vi "Correlation_Contrast_Tau_Manipulation.vi"(8 "Numeric 2":i32, 9 "Dont invert?":bool, 10 "Numeric":i32, 11 "MW Step Size":dbl=2e-09) -> (3 "Tau":dbl)   [LabVIEW 2024]
uses:
  <vilib>/Utility/error.llb/DialogTypeEnum.ctl
  SpinCore_API_file_location.vi
panel:
  in  "# of Instructions":u32=89
  in  "Instructions":T1(array[cluster])=[{"Instruct Data"=0, "Op Code"=0, "Flags"=[FALSE, FALSE, TRUE, FALSE, FALSE, FALSE, FALSE, TRUE, FALSE, FALSE, FALSE, FALSE, FALSE, FALSE, FALSE, FALSE, FALSE, FALSE, FALSE, FALSE, FALSE, FALSE, FALSE, TRUE], "Comments"="0 Triggers", "Time (s)"=1e-07}, {"Instruct Data"=0, "Op Code"=0, "Flags"=[FALSE, FALSE, FALSE, FALSE, FALSE, FALSE, FALSE, TRUE, FALSE, FALSE, FALSE, FALSE, FALSE, FALSE, FALSE, FALSE, FALSE, FALSE, FALSE, FALSE, FALSE, FALSE, FALSE, FALSE], "Comments"="1 Dark ", "Time (s)"=1e-05}, {"Instruct Data"=0, "Op Code"=0, "Flags"=[FALSE, FALSE, FALSE, FALSE, FALSE, FALSE, FALSE, TRUE, FALSE, FALSE, FALSE, FALSE, FALSE, FALSE, FALSE, FALSE, FALSE, FALSE, FALSE, FALSE, FALSE, FALSE, FALSE, FALSE], "Comments"="2 AOM Buffer", "Time (s)"=5e-07}, {"Instruct Data"=0, "Op Code"=0, "Flags"=[TRUE, FALSE, FALSE, TRUE, FALSE, FALSE, FALSE, TRUE, FALSE, FALSE, FALSE, FALSE, FALSE, FALSE, FALSE, FALSE, FALSE, FALSE, FALSE, FALSE, FALSE, FALSE, FALSE, FALSE], "Comments"="3 pi/2_X", "Time (s)"=3.7e-08}, {"Instruct Data"=0, "Op Code"=0, "Flags"=[FALSE, FALSE, FALSE, FALSE, FALSE, FALSE, FALSE, TRUE, FALSE, FALSE, FALSE, FALSE, FALSE, FALSE, FALSE, FALSE, FALSE, FALSE, FALSE, FALSE, FALSE, FALSE, FALSE, FALSE], "Comments"="4 tau/2", "Time (s)"=2.105e-06}, {"Instruct Data"=0, "Op Code"=0, "Flags"=[TRUE, FALSE, FALSE, TRUE, FALSE, FALSE, FALSE, TRUE, FALSE, FALSE, FALSE, FALSE, FALSE, FALSE, FALSE, FALSE, FALSE, FALSE, FALSE, FALSE, FALSE, FALSE, FALSE, FALSE], "Comments"="5  Pi_X", "Time (s)"=6.7e-08}, {"Instruct Data"=0, "Op Code"=0, "Flags"=[FALSE, FALSE, FALSE, FALSE, FALSE, FALSE, FALSE, TRUE, FALSE, FALSE, FALSE, FALSE, FALSE, FALSE, FALSE, FALSE, FALSE, FALSE, FALSE, FALSE, FALSE, FALSE, FALSE, FALSE], "Comments"="6 Tau", "Time (s)"=4.21e-06}, {"Instruct Data"=0, "Op Code"=0, "Flags"=[TRUE, FALSE, FALSE, FALSE, TRUE, FALSE, FALSE, TRUE, FALSE, FALSE, FALSE, FALSE, FALSE, FALSE, FALSE, FALSE, FALSE, FALSE, FALSE, FALSE, FALSE, FALSE, FALSE, FALSE], "Comments"="7 Pi_Y", "Time (s)"=7e-08}, {"Instruct Data"=0, "Op Code"=0, "Flags"=[FALSE, FALSE, FALSE, FALSE, FALSE, FALSE, FALSE, TRUE, FALSE, FALSE, FALSE, FALSE, FALSE, FALSE, FALSE, FALSE, FALSE, FALSE, FALSE, FALSE, FALSE, FALSE, FALSE, FALSE], "Comments"="8 Tau", "Time (s)"=4.21e-06}, {"Instruct Data"=0, "Op Code"=0, "Flags"=[TRUE, FALSE, FALSE, TRUE, FALSE, FALSE, FALSE, TRUE, FALSE, FALSE, FALSE, FALSE, FALSE, FALSE, FALSE, FALSE, FALSE, FALSE, FALSE, FALSE, FALSE, FALSE, FALSE, FALSE], "Comments"="9 Pi_X", "Time (s)"=6.7e-08}, {"Instruct Data"=0, "Op Code"=0, "Flags"=[FALSE, FALSE, FALSE, FALSE, FALSE, FALSE, FALSE, TRUE, FALSE, FALSE, FALSE, FALSE, FALSE, FALSE, FALSE, FALSE, FALSE, FALSE, FALSE, FALSE, FALSE, FALSE, FALSE, FALSE], "Comments"="10 tau", "Time (s)"=4.21e-06}, {"Instruct Data"=0, "Op Code"=0, "Flags"=[TRUE, FALSE, FALSE, FALSE, TRUE, FALSE, FALSE, TRUE, FALSE, FALSE, FALSE, FALSE, FALSE, FALSE, FALSE, FALSE, FALSE, FALSE, FALSE, FALSE, FALSE, FALSE, FALSE, FALSE], "Comments"="11 Pi_Y", "Time (s)"=7e-08}, {"Instruct Data"=0, "Op Code"=0, "Flags"=[FALSE, FALSE, FALSE, FALSE, FALSE, FALSE, FALSE, TRUE, FALSE, FALSE, FALSE, FALSE, FALSE, FALSE, FALSE, FALSE, FALSE, FALSE, FALSE, FALSE, FALSE, FALSE, FALSE, FALSE], "Comments"="12 Tau", "Time (s)"=4.21e-06}, {"Instruct Data"=0, "Op Code"=0, "Flags"=[TRUE, FALSE, FALSE, FALSE, TRUE, FALSE, FALSE, TRUE, FALSE, FALSE, FALSE, FALSE, FALSE, FALSE, FALSE, FALSE, FALSE, FALSE, FALSE, FALSE, FALSE, FALSE, FALSE, FALSE], "Comments"="13 Pi_Y", "Time (s)"=7e-08}, {"Instruct Data"=0, "Op Code"=0, "Flags"=[FALSE, FALSE, FALSE, FALSE, FALSE, FALSE, FALSE, TRUE, FALSE, FALSE, FALSE, FALSE, FALSE, FALSE, FALSE, FALSE, FALSE, FALSE, FALSE, FALSE, FALSE, FALSE, FALSE, FALSE], "Comments"="14 tau", "Time (s)"=4.21e-06}, {"Instruct Data"=0, "Op Code"=0, "Flags"=[TRUE, FALSE, FALSE, TRUE, FALSE, FALSE, FALSE, TRUE, FALSE, FALSE, FALSE, FALSE, FALSE, FALSE, FALSE, FALSE, FALSE, FALSE, FALSE, FALSE, FALSE, FALSE, FALSE, FALSE], "Comments"="15 Pi_X", "Time (s)"=6.7e-08}, {"Instruct Data"=0, "Op Code"=0, "Flags"=[FALSE, FALSE, FALSE, FALSE, FALSE, FALSE, FALSE, TRUE, FALSE, FALSE, FALSE, FALSE, FALSE, FALSE, FALSE, FALSE, FALSE, FALSE, FALSE, FALSE, FALSE, FALSE, FALSE, FALSE], "Comments"="16  tau", "Time (s)"=4.21e-06}, {"Instruct Data"=0, "Op Code"=0, "Flags"=[TRUE, FALSE, FALSE, FALSE, TRUE, FALSE, FALSE, TRUE, FALSE, FALSE, FALSE, FALSE, FALSE, FALSE, FALSE, FALSE, FALSE, FALSE, FALSE, FALSE, FALSE, FALSE, FALSE, FALSE], "Comments"="17 Pi_Y", "Time (s)"=7e-08}, {"Instruct Data"=0, "Op Code"=0, "Flags"=[FALSE, FALSE, FALSE, FALSE, FALSE, FALSE, FALSE, TRUE, FALSE, FALSE, FALSE, FALSE, FALSE, FALSE, FALSE, FALSE, FALSE, FALSE, FALSE, FALSE, FALSE, FALSE, FALSE, FALSE], "Comments"="18 tau", "Time (s)"=4.21e-06}, {"Instruct Data"=0, "Op Code"=0, "Flags"=[TRUE, FALSE, FALSE, TRUE, FALSE, FALSE, FALSE, TRUE, FALSE, FALSE, FALSE, FALSE, FALSE, FALSE, FALSE, FALSE, FALSE, FALSE, FALSE, FALSE, FALSE, FALSE, FALSE, FALSE], "Comments"="19 pi_X", "Time (s)"=6.7e-08}, {"Instruct Data"=0, "Op Code"=0, "Flags"=[FALSE, FALSE, FALSE, FALSE, FALSE, FALSE, FALSE, TRUE, FALSE, FALSE, FALSE, FALSE, FALSE, FALSE, FALSE, FALSE, FALSE, FALSE, FALSE, FALSE, FALSE, FALSE, FALSE, FALSE], "Comments"="20  tau/2", "Time (s)"=2.105e-06}, {"Instruct Data"=0, "Op Code"=0, "Flags"=[TRUE, FALSE, FALSE, FALSE, TRUE, FALSE, FALSE, TRUE, FALSE, FALSE, FALSE, FALSE, FALSE, FALSE, FALSE, FALSE, FALSE, FALSE, FALSE, FALSE, FALSE, FALSE, FALSE, FALSE], "Comments"="21 pi/2_Y", "Time (s)"=3.9e-08}, {"Instruct Data"=0, "Op Code"=0, "Flags"=[FALSE, FALSE, FALSE, FALSE, FALSE, FALSE, FALSE, TRUE, FALSE, FALSE, FALSE, FALSE, FALSE, FALSE, FALSE, FALSE, FALSE, FALSE, FALSE, FALSE, FALSE, FALSE, FALSE, FALSE], "Comments"="22 CC tau", "Time (s)"=1e-08}, {"Instruct Data"=0, "Op Code"=0, "Flags"=[TRUE, FALSE, FALSE, TRUE, FALSE, FALSE, FALSE, TRUE, FALSE, FALSE, FALSE, FALSE, FALSE, FALSE, FALSE, FALSE, FALSE, FALSE, FALSE, FALSE, FALSE, FALSE, FALSE, FALSE], "Comments"="23  pi/2_X", "Time (s)"=3.7e-08}, {"Instruct Data"=0, "Op Code"=0, "Flags"=[FALSE, FALSE, FALSE, FALSE, FALSE, FALSE, FALSE, TRUE, FALSE, FALSE, FALSE, FALSE, FALSE, FALSE, FALSE, FALSE, FALSE, FALSE, FALSE, FALSE, FALSE, FALSE, FALSE, FALSE], "Comments"="24  tau/2", "Time (s)"=2.105e-06}, {"Instruct Data"=0, "Op Code"=0, "Flags"=[TRUE, FALSE, FALSE, TRUE, FALSE, FALSE, FALSE, TRUE, FALSE, FALSE, FALSE, FALSE, FALSE, FALSE, FALSE, FALSE, FALSE, FALSE, FALSE, FALSE, FALSE, FALSE, FALSE, FALSE], "Comments"="25  pi_X", "Time (s)"=6.7e-08}, {"Instruct Data"=0, "Op Code"=0, "Flags"=[FALSE, FALSE, FALSE, FALSE, FALSE, FALSE, FALSE, TRUE, FALSE, FALSE, FALSE, FALSE, FALSE, FALSE, FALSE, FALSE, FALSE, FALSE, FALSE, FALSE, FALSE, FALSE, FALSE, FALSE], "Comments"="26  tau", "Time (s)"=4.21e-06}, {"Instruct Data"=0, "Op Code"=0, "Flags"=[TRUE, FALSE, FALSE, FALSE, TRUE, FALSE, FALSE, TRUE, FALSE, FALSE, FALSE, FALSE, FALSE, FALSE, FALSE, FALSE, FALSE, FALSE, FALSE, FALSE, FALSE, FALSE, FALSE, FALSE], "Comments"="27  pi_Y", "Time (s)"=7e-08}, {"Instruct Data"=0, "Op Code"=0, "Flags"=[FALSE, FALSE, FALSE, FALSE, FALSE, FALSE, FALSE, TRUE, FALSE, FALSE, FALSE, FALSE, FALSE, FALSE, FALSE, FALSE, FALSE, FALSE, FALSE, FALSE, FALSE, FALSE, FALSE, FALSE], "Comments"="28  tau", "Time (s)"=4.21e-06}, {"Instruct Data"=0, "Op Code"=0, "Flags"=[TRUE, FALSE, FALSE, TRUE, FALSE, FALSE, FALSE, TRUE, FALSE, FALSE, FALSE, FALSE, FALSE, FALSE, FALSE, FALSE, FALSE, FALSE, FALSE, FALSE, FALSE, FALSE, FALSE, FALSE], "Comments"="29  Pi_X", "Time (s)"=6.7e-08}, {"Instruct Data"=0, "Op Code"=0, "Flags"=[FALSE, FALSE, FALSE, FALSE, FALSE, FALSE, FALSE, TRUE, FALSE, FALSE, FALSE, FALSE, FALSE, FALSE, FALSE, FALSE, FALSE, FALSE, FALSE, FALSE, FALSE, FALSE, FALSE, FALSE], "Comments"="30  tau", "Time (s)"=4.21e-06}, {"Instruct Data"=0, "Op Code"=0, "Flags"=[TRUE, FALSE, FALSE, FALSE, TRUE, FALSE, FALSE, TRUE, FALSE, FALSE, FALSE, FALSE, FALSE, FALSE, FALSE, FALSE, FALSE, FALSE, FALSE, FALSE, FALSE, FALSE, FALSE, FALSE], "Comments"="31  Pi_y", "Time (s)"=7e-08}, {"Instruct Data"=0, "Op Code"=0, "Flags"=[FALSE, FALSE, FALSE, FALSE, FALSE, FALSE, FALSE, TRUE, FALSE, FALSE, FALSE, FALSE, FALSE, FALSE, FALSE, FALSE, FALSE, FALSE, FALSE, FALSE, FALSE, FALSE, FALSE, FALSE], "Comments"="32  tau", "Time (s)"=4.21e-06}, {"Instruct Data"=0, "Op Code"=0, "Flags"=[TRUE, FALSE, FALSE, FALSE, TRUE, FALSE, FALSE, TRUE, FALSE, FALSE, FALSE, FALSE, FALSE, FALSE, FALSE, FALSE, FALSE, FALSE, FALSE, FALSE, FALSE, FALSE, FALSE, FALSE], "Comments"="33  Pi_Y", "Time (s)"=7e-08}, {"Instruct Data"=0, "Op Code"=0, "Flags"=[FALSE, FALSE, FALSE, FALSE, FALSE, FALSE, FALSE, TRUE, FALSE, FALSE, FALSE, FALSE, FALSE, FALSE, FALSE, FALSE, FALSE, FALSE, FALSE, FALSE, FALSE, FALSE, FALSE, FALSE], "Comments"="34  tau", "Time (s)"=4.21e-06}, {"Instruct Data"=0, "Op Code"=0, "Flags"=[TRUE, FALSE, FALSE, TRUE, FALSE, FALSE, FALSE, TRUE, FALSE, FALSE, FALSE, FALSE, FALSE, FALSE, FALSE, FALSE, FALSE, FALSE, FALSE, FALSE, FALSE, FALSE, FALSE, FALSE], "Comments"="35 Pi_X", "Time (s)"=6.7e-08}, {"Instruct Data"=0, "Op Code"=0, "Flags"=[FALSE, FALSE, FALSE, FALSE, FALSE, FALSE, FALSE, TRUE, FALSE, FALSE, FALSE, FALSE, FALSE, FALSE, FALSE, FALSE, FALSE, FALSE, FALSE, FALSE, FALSE, FALSE, FALSE, FALSE], "Comments"="36  tau", "Time (s)"=4.21e-06}, {"Instruct Data"=0, "Op Code"=0, "Flags"=[TRUE, FALSE, FALSE, FALSE, TRUE, FALSE, FALSE, TRUE, FALSE, FALSE, FALSE, FALSE, FALSE, FALSE, FALSE, FALSE, FALSE, FALSE, FALSE, FALSE, FALSE, FALSE, FALSE, FALSE], "Comments"="37  Pi_Y", "Time (s)"=7e-08}, {"Instruct Data"=0, "Op Code"=0, "Flags"=[FALSE, FALSE, FALSE, FALSE, FALSE, FALSE, FALSE, TRUE, FALSE, FALSE, FALSE, FALSE, FALSE, FALSE, FALSE, FALSE, FALSE, FALSE, FALSE, FALSE, FALSE, FALSE, FALSE, FALSE], "Comments"="38  tau", "Time (s)"=4.21e-06}, {"Instruct Data"=0, "Op Code"=0, "Flags"=[TRUE, FALSE, FALSE, TRUE, FALSE, FALSE, FALSE, TRUE, FALSE, FALSE, FALSE, FALSE, FALSE, FALSE, FALSE, FALSE, FALSE, FALSE, FALSE, FALSE, FALSE, FALSE, FALSE, FALSE], "Comments"="39  Pi_X", "Time (s)"=6.7e-08}, {"Instruct Data"=0, "Op Code"=0, "Flags"=[FALSE, FALSE, FALSE, FALSE, FALSE, FALSE, FALSE, TRUE, FALSE, FALSE, FALSE, FALSE, FALSE, FALSE, FALSE, FALSE, FALSE, FALSE, FALSE, FALSE, FALSE, FALSE, FALSE, FALSE], "Comments"="40  tau/2", "Time (s)"=2.105e-06}, {"Instruct Data"=0, "Op Code"=0, "Flags"=[TRUE, FALSE, FALSE, FALSE, TRUE, FALSE, FALSE, TRUE, FALSE, FALSE, FALSE, FALSE, FALSE, FALSE, FALSE, FALSE, FALSE, FALSE, FALSE, FALSE, FALSE, FALSE, FALSE, FALSE], "Comments"="41  pi/2_Y", "Time (s)"=3.9e-08}, {"Instruct Data"=0, "Op Code"=0, "Flags"=[FALSE, TRUE, FALSE, FALSE, FALSE, FALSE, FALSE, TRUE, FALSE, FALSE, FALSE, FALSE, FALSE, FALSE, FALSE, FALSE, FALSE, FALSE, FALSE, FALSE, FALSE, FALSE, FALSE, FALSE], "Comments"="42  AOM Buffer", "Time (s)"=5e-07}, {"Instruct Data"=0, "Op Code"=0, "Flags"=[FALSE, TRUE, FALSE, FALSE, FALSE, FALSE, FALSE, FALSE, FALSE, FALSE, FALSE, FALSE, FALSE, FALSE, FALSE, FALSE, FALSE, FALSE, FALSE, FALSE, FALSE, FALSE, FALSE, FALSE], "Comments"="43  inhibit off", "Time (s)"=5e-07}, {"Instruct Data"=0, "Op Code"=0, "Flags"=[FALSE, TRUE, FALSE, FALSE, FALSE, FALSE, FALSE, TRUE, FALSE, FALSE, FALSE, FALSE, FALSE, FALSE, FALSE, FALSE, FALSE, FALSE, FALSE, FALSE, FALSE, FALSE, FALSE, FALSE], "Comments"="44  AOM", "Time (s)"=5e-06}, {"Instruct Data"=0, "Op Code"=0, "Flags"=[FALSE, FALSE, FALSE, FALSE, FALSE, FALSE, FALSE, TRUE, FALSE, FALSE, FALSE, FALSE, FALSE, FALSE, FALSE, FALSE, FALSE, FALSE, FALSE, FALSE, FALSE, FALSE, FALSE, FALSE], "Comments"="45  AOM buffer", "Time (s)"=5e-07}, {"Instruct Data"=0, "Op Code"=0, "Flags"=[FALSE, FALSE, FALSE, FALSE, FALSE, FALSE, FALSE, TRUE, FALSE, FALSE, FALSE, FALSE, FALSE, FALSE, FALSE, FALSE, FALSE, FALSE, FALSE, FALSE, FALSE, FALSE, FALSE, FALSE], "Comments"="46  Dark", "Time (s)"=1e-05}, {"Instruct Data"=0, "Op Code"=0, "Flags"=[TRUE, FALSE, FALSE, TRUE, FALSE, FALSE, FALSE, TRUE, FALSE, FALSE, FALSE, FALSE, FALSE, FALSE, FALSE, FALSE, FALSE, FALSE, FALSE, FALSE, FALSE, FALSE, FALSE, FALSE], "Comments"="47  pi/2_X", "Time (s)"=3.6e-08}, {"Instruct Data"=0, "Op Code"=0, "Flags"=[FALSE, FALSE, FALSE, FALSE, FALSE, FALSE, FALSE, TRUE, FALSE, FALSE, FALSE, FALSE, FALSE, FALSE, FALSE, FALSE, FALSE, FALSE, FALSE, FALSE, FALSE, FALSE, FALSE, FALSE], "Comments"="48  tau/2", "Time (s)"=2.105e-06}, {"Instruct Data"=0, "Op Code"=0, "Flags"=[TRUE, FALSE, FALSE, TRUE, FALSE, FALSE, FALSE, TRUE, FALSE, FALSE, FALSE, FALSE, FALSE, FALSE, FALSE, FALSE, FALSE, FALSE, FALSE, FALSE, FALSE, FALSE, FALSE, FALSE], "Comments"="49 Pi_X", "Time (s)"=6.7e-08}, {"Instruct Data"=0, "Op Code"=0, "Flags"=[FALSE, FALSE, FALSE, FALSE, FALSE, FALSE, FALSE, TRUE, FALSE, FALSE, FALSE, FALSE, FALSE, FALSE, FALSE, FALSE, FALSE, FALSE, FALSE, FALSE, FALSE, FALSE, FALSE, FALSE], "Comments"="50 tau", "Time (s)"=4.21e-06}, {"Instruct Data"=0, "Op Code"=0, "Flags"=[TRUE, FALSE, FALSE, FALSE, TRUE, FALSE, FALSE, TRUE, FALSE, FALSE, FALSE, FALSE, FALSE, FALSE, FALSE, FALSE, FALSE, FALSE, FALSE, FALSE, FALSE, FALSE, FALSE, FALSE], "Comments"="51 Pi_y", "Time (s)"=7e-08}, {"Instruct Data"=0, "Op Code"=0, "Flags"=[FALSE, FALSE, FALSE, FALSE, FALSE, FALSE, FALSE, TRUE, FALSE, FALSE, FALSE, FALSE, FALSE, FALSE, FALSE, FALSE, FALSE, FALSE, FALSE, FALSE, FALSE, FALSE, FALSE, FALSE], "Comments"="52 tau", "Time (s)"=4.21e-06}, {"Instruct Data"=0, "Op Code"=0, "Flags"=[TRUE, FALSE, FALSE, TRUE, FALSE, FALSE, FALSE, TRUE, FALSE, FALSE, FALSE, FALSE, FALSE, FALSE, FALSE, FALSE, FALSE, FALSE, FALSE, FALSE, FALSE, FALSE, FALSE, FALSE], "Comments"="53 pi_x", "Time (s)"=6.7e-08}, {"Instruct Data"=0, "Op Code"=0, "Flags"=[FALSE, FALSE, FALSE, FALSE, FALSE, FALSE, FALSE, TRUE, FALSE, FALSE, FALSE, FALSE, FALSE, FALSE, FALSE, FALSE, FALSE, FALSE, FALSE, FALSE, FALSE, FALSE, FALSE, FALSE], "Comments"="54 tau", "Time (s)"=4.21e-06}, {"Instruct Data"=0, "Op Code"=0, "Flags"=[TRUE, FALSE, FALSE, FALSE, TRUE, FALSE, FALSE, TRUE, FALSE, FALSE, FALSE, FALSE, FALSE, FALSE, FALSE, FALSE, FALSE, FALSE, FALSE, FALSE, FALSE, FALSE, FALSE, FALSE], "Comments"="55 Pi_Y", "Time (s)"=7e-08}, {"Instruct Data"=0, "Op Code"=0, "Flags"=[FALSE, FALSE, FALSE, FALSE, FALSE, FALSE, FALSE, TRUE, FALSE, FALSE, FALSE, FALSE, FALSE, FALSE, FALSE, FALSE, FALSE, FALSE, FALSE, FALSE, FALSE, FALSE, FALSE, FALSE], "Comments"="56 tau", "Time (s)"=4.21e-06}, {"Instruct Data"=0, "Op Code"=0, "Flags"=[TRUE, FALSE, FALSE, FALSE, TRUE, FALSE, FALSE, TRUE, FALSE, FALSE, FALSE, FALSE, FALSE, FALSE, FALSE, FALSE, FALSE, FALSE, FALSE, FALSE, FALSE, FALSE, FALSE, FALSE], "Comments"="57 Pi_y", "Time (s)"=7e-08}, {"Instruct Data"=0, "Op Code"=0, "Flags"=[FALSE, FALSE, FALSE, FALSE, FALSE, FALSE, FALSE, TRUE, FALSE, FALSE, FALSE, FALSE, FALSE, FALSE, FALSE, FALSE, FALSE, FALSE, FALSE, FALSE, FALSE, FALSE, FALSE, FALSE], "Comments"="58 tau", "Time (s)"=4.21e-06}, {"Instruct Data"=0, "Op Code"=0, "Flags"=[TRUE, FALSE, FALSE, TRUE, FALSE, FALSE, FALSE, TRUE, FALSE, FALSE, FALSE, FALSE, FALSE, FALSE, FALSE, FALSE, FALSE, FALSE, FALSE, FALSE, FALSE, FALSE, FALSE, FALSE], "Comments"="59 Pi_x", "Time (s)"=6.7e-08}, {"Instruct Data"=0, "Op Code"=0, "Flags"=[FALSE, FALSE, FALSE, FALSE, FALSE, FALSE, FALSE, TRUE, FALSE, FALSE, FALSE, FALSE, FALSE, FALSE, FALSE, FALSE, FALSE, FALSE, FALSE, FALSE, FALSE, FALSE, FALSE, FALSE], "Comments"="60 tau", "Time (s)"=4.21e-06}, {"Instruct Data"=0, "Op Code"=0, "Flags"=[TRUE, FALSE, FALSE, FALSE, TRUE, FALSE, FALSE, TRUE, FALSE, FALSE, FALSE, FALSE, FALSE, FALSE, FALSE, FALSE, FALSE, FALSE, FALSE, FALSE, FALSE, FALSE, FALSE, FALSE], "Comments"="61 Pi_y", "Time (s)"=7e-08}, {"Instruct Data"=0, "Op Code"=0, "Flags"=[FALSE, FALSE, FALSE, FALSE, FALSE, FALSE, FALSE, TRUE, FALSE, FALSE, FALSE, FALSE, FALSE, FALSE, FALSE, FALSE, FALSE, FALSE, FALSE, FALSE, FALSE, FALSE, FALSE, FALSE], "Comments"="62 tau", "Time (s)"=4.21e-06}, {"Instruct Data"=0, "Op Code"=0, "Flags"=[TRUE, FALSE, FALSE, TRUE, FALSE, FALSE, FALSE, TRUE, FALSE, FALSE, FALSE, FALSE, FALSE, FALSE, FALSE, FALSE, FALSE, FALSE, FALSE, FALSE, FALSE, FALSE, FALSE, FALSE], "Comments"="63 pi_X", "Time (s)"=6.7e-08}, {"Instruct Data"=0, "Op Code"=0, "Flags"=[FALSE, FALSE, FALSE, FALSE, FALSE, FALSE, FALSE, TRUE, FALSE, FALSE, FALSE, FALSE, FALSE, FALSE, FALSE, FALSE, FALSE, FALSE, FALSE, FALSE, FALSE, FALSE, FALSE, FALSE], "Comments"="64 Tau /2", "Time (s)"=2.105e-06}, {"Instruct Data"=0, "Op Code"=0, "Flags"=[TRUE, FALSE, FALSE, FALSE, TRUE, FALSE, FALSE, TRUE, FALSE, FALSE, FALSE, FALSE, FALSE, FALSE, FALSE, FALSE, FALSE, FALSE, FALSE, FALSE, FALSE, FALSE, FALSE, FALSE], "Comments"="65 pi/2_Y", "Time (s)"=3.8e-08}, {"Instruct Data"=0, "Op Code"=0, "Flags"=[FALSE, FALSE, FALSE, FALSE, FALSE, FALSE, FALSE, TRUE, FALSE, FALSE, FALSE, FALSE, FALSE, FALSE, FALSE, FALSE, FALSE, FALSE, FALSE, FALSE, FALSE, FALSE, FALSE, FALSE], "Comments"="66  TAU CC", "Time (s)"=1e-08}, {"Instruct Data"=0, "Op Code"=0, "Flags"=[TRUE, FALSE, FALSE, TRUE, FALSE, FALSE, FALSE, TRUE, FALSE, FALSE, FALSE, FALSE, FALSE, FALSE, FALSE, FALSE, FALSE, FALSE, FALSE, FALSE, FALSE, FALSE, FALSE, FALSE], "Comments"="67 pi/2_X", "Time (s)"=3.7e-08}, {"Instruct Data"=0, "Op Code"=0, "Flags"=[FALSE, FALSE, FALSE, FALSE, FALSE, FALSE, FALSE, TRUE, FALSE, FALSE, FALSE, FALSE, FALSE, FALSE, FALSE, FALSE, FALSE, FALSE, FALSE, FALSE, FALSE, FALSE, FALSE, FALSE], "Comments"="68 tau/2", "Time (s)"=2.105e-06}, {"Instruct Data"=0, "Op Code"=0, "Flags"=[TRUE, FALSE, FALSE, TRUE, FALSE, FALSE, FALSE, TRUE, FALSE, FALSE, FALSE, FALSE, FALSE, FALSE, FALSE, FALSE, FALSE, FALSE, FALSE, FALSE, FALSE, FALSE, FALSE, FALSE], "Comments"="69 Pi_x", "Time (s)"=6.7e-08}, {"Instruct Data"=0, "Op Code"=0, "Flags"=[FALSE, FALSE, FALSE, FALSE, FALSE, FALSE, FALSE, TRUE, FALSE, FALSE, FALSE, FALSE, FALSE, FALSE, FALSE, FALSE, FALSE, FALSE, FALSE, FALSE, FALSE, FALSE, FALSE, FALSE], "Comments"="70 tau", "Time (s)"=4.21e-06}, {"Instruct Data"=0, "Op Code"=0, "Flags"=[TRUE, FALSE, FALSE, FALSE, TRUE, FALSE, FALSE, TRUE, FALSE, FALSE, FALSE, FALSE, FALSE, FALSE, FALSE, FALSE, FALSE, FALSE, FALSE, FALSE, FALSE, FALSE, FALSE, FALSE], "Comments"="71 Pi_y", "Time (s)"=7e-08}, {"Instruct Data"=0, "Op Code"=0, "Flags"=[FALSE, FALSE, FALSE, FALSE, FALSE, FALSE, FALSE, TRUE, FALSE, FALSE, FALSE, FALSE, FALSE, FALSE, FALSE, FALSE, FALSE, FALSE, FALSE, FALSE, FALSE, FALSE, FALSE, FALSE], "Comments"="72 tau", "Time (s)"=4.21e-06}, {"Instruct Data"=0, "Op Code"=0, "Flags"=[TRUE, FALSE, FALSE, TRUE, FALSE, FALSE, FALSE, TRUE, FALSE, FALSE, FALSE, FALSE, FALSE, FALSE, FALSE, FALSE, FALSE, FALSE, FALSE, FALSE, FALSE, FALSE, FALSE, FALSE], "Comments"="73 Pi_x", "Time (s)"=6.7e-08}, {"Instruct Data"=0, "Op Code"=0, "Flags"=[FALSE, FALSE, FALSE, FALSE, FALSE, FALSE, FALSE, TRUE, FALSE, FALSE, FALSE, FALSE, FALSE, FALSE, FALSE, FALSE, FALSE, FALSE, FALSE, FALSE, FALSE, FALSE, FALSE, FALSE], "Comments"="74 tau", "Time (s)"=4.21e-06}, {"Instruct Data"=0, "Op Code"=0, "Flags"=[TRUE, FALSE, FALSE, FALSE, TRUE, FALSE, FALSE, TRUE, FALSE, FALSE, FALSE, FALSE, FALSE, FALSE, FALSE, FALSE, FALSE, FALSE, FALSE, FALSE, FALSE, FALSE, FALSE, FALSE], "Comments"="75 Pi_Y", "Time (s)"=7e-08}, {"Instruct Data"=0, "Op Code"=0, "Flags"=[FALSE, FALSE, FALSE, FALSE, FALSE, FALSE, FALSE, TRUE, FALSE, FALSE, FALSE, FALSE, FALSE, FALSE, FALSE, FALSE, FALSE, FALSE, FALSE, FALSE, FALSE, FALSE, FALSE, FALSE], "Comments"="76 tau ", "Time (s)"=4.21e-06}, {"Instruct Data"=0, "Op Code"=0, "Flags"=[TRUE, FALSE, FALSE, FALSE, TRUE, FALSE, FALSE, TRUE, FALSE, FALSE, FALSE, FALSE, FALSE, FALSE, FALSE, FALSE, FALSE, FALSE, FALSE, FALSE, FALSE, FALSE, FALSE, FALSE], "Comments"="77 Pi_y", "Time (s)"=7e-08}, {"Instruct Data"=0, "Op Code"=0, "Flags"=[FALSE, FALSE, FALSE, FALSE, FALSE, FALSE, FALSE, TRUE, FALSE, FALSE, FALSE, FALSE, FALSE, FALSE, FALSE, FALSE, FALSE, FALSE, FALSE, FALSE, FALSE, FALSE, FALSE, FALSE], "Comments"="78 tau", "Time (s)"=4.21e-06}, {"Instruct Data"=0, "Op Code"=0, "Flags"=[TRUE, FALSE, FALSE, TRUE, FALSE, FALSE, FALSE, TRUE, FALSE, FALSE, FALSE, FALSE, FALSE, FALSE, FALSE, FALSE, FALSE, FALSE, FALSE, FALSE, FALSE, FALSE, FALSE, FALSE], "Comments"="79 Pi_x", "Time (s)"=6.7e-08}, {"Instruct Data"=0, "Op Code"=0, "Flags"=[FALSE, FALSE, FALSE, FALSE, FALSE, FALSE, FALSE, TRUE, FALSE, FALSE, FALSE, FALSE, FALSE, FALSE, FALSE, FALSE, FALSE, FALSE, FALSE, FALSE, FALSE, FALSE, FALSE, FALSE], "Comments"="80 tau", "Time (s)"=4.21e-06}, {"Instruct Data"=0, "Op Code"=0, "Flags"=[TRUE, FALSE, FALSE, FALSE, TRUE, FALSE, FALSE, TRUE, FALSE, FALSE, FALSE, FALSE, FALSE, FALSE, FALSE, FALSE, FALSE, FALSE, FALSE, FALSE, FALSE, FALSE, FALSE, FALSE], "Comments"="81 Pi_y", "Time (s)"=7e-08}, {"Instruct Data"=0, "Op Code"=0, "Flags"=[FALSE, FALSE, FALSE, FALSE, FALSE, FALSE, FALSE, TRUE, FALSE, FALSE, FALSE, FALSE, FALSE, FALSE, FALSE, FALSE, FALSE, FALSE, FALSE, FALSE, FALSE, FALSE, FALSE, FALSE], "Comments"="82 tau", "Time (s)"=4.21e-06}, {"Instruct Data"=0, "Op Code"=0, "Flags"=[TRUE, FALSE, FALSE, TRUE, FALSE, FALSE, FALSE, TRUE, FALSE, FALSE, FALSE, FALSE, FALSE, FALSE, FALSE, FALSE, FALSE, FALSE, FALSE, FALSE, FALSE, FALSE, FALSE, FALSE], "Comments"="83 Pi_X", "Time (s)"=6.7e-08}, {"Instruct Data"=0, "Op Code"=0, "Flags"=[FALSE, FALSE, FALSE, FALSE, FALSE, FALSE, FALSE, TRUE, FALSE, FALSE, FALSE, FALSE, FALSE, FALSE, FALSE, FALSE, FALSE, FALSE, FALSE, FALSE, FALSE, FALSE, FALSE, FALSE], "Comments"="84 tau/2", "Time (s)"=2.105e-06}, {"Instruct Data"=0, "Op Code"=0, "Flags"=[TRUE, FALSE, FALSE, FALSE, TRUE, FALSE, FALSE, TRUE, FALSE, FALSE, FALSE, FALSE, FALSE, FALSE, FALSE, FALSE, FALSE, FALSE, FALSE, FALSE, FALSE, FALSE, FALSE, FALSE], "Comments"="85 3pi/2_Y", "Time (s)"=1.05e-07}, {"Instruct Data"=0, "Op Code"=0, "Flags"=[FALSE, TRUE, FALSE, FALSE, FALSE, FALSE, FALSE, TRUE, FALSE, FALSE, FALSE, FALSE, FALSE, FALSE, FALSE, FALSE, FALSE, FALSE, FALSE, FALSE, FALSE, FALSE, FALSE, FALSE], "Comments"="86 AOM delay", "Time (s)"=5e-07}, {"Instruct Data"=0, "Op Code"=0, "Flags"=[FALSE, TRUE, FALSE, FALSE, FALSE, FALSE, FALSE, FALSE, FALSE, FALSE, FALSE, FALSE, FALSE, FALSE, FALSE, FALSE, FALSE, FALSE, FALSE, FALSE, FALSE, FALSE, FALSE, FALSE], "Comments"="87 Inhibit off", "Time (s)"=5e-07}, {"Instruct Data"=0, "Op Code"=6, "Flags"=[FALSE, TRUE, FALSE, FALSE, FALSE, FALSE, FALSE, TRUE, FALSE, FALSE, FALSE, FALSE, FALSE, FALSE, FALSE, FALSE, FALSE, FALSE, FALSE, FALSE, FALSE, FALSE, FALSE, FALSE], "Comments"="88 AOM", "Time (s)"=5e-06}] {"Time (s)" format="%.3p"; "Op Code" items=["Continue", "Stop", "Loop", "End Loop", "JSR", "RTS", "Branch", "Long Delay", "Wait"]}
  out "output array":T1(array[cluster])
  in  "clock_freq (MHz)":dbl=500.0
  out "x+y 2":dbl
  out "x+y 3":dbl
  out "x+y 4":dbl
  out "output array 2":T1(array[cluster])
  in  "clock_freq (MHz) 2":dbl=500.0
  out "x+y 11":dbl
  out "x+y 10":dbl
  out "x+y 9":dbl
  # "4.210u"
  # "22"
  # "here"
  # "66"
  # "1"
  # "2"
  # "3"
  # "4"
  # "5"
  # "6"
  # "7"
  # "8"
  # "9"
  # "10"
  # "11"
  # "12"
  # "13"
  # "14"
  # "15"
  # "16"
  # "17"
  # "18"
  # "19"
  # "20"
  # "21"
  # "22"
  # "23"
  # "24"
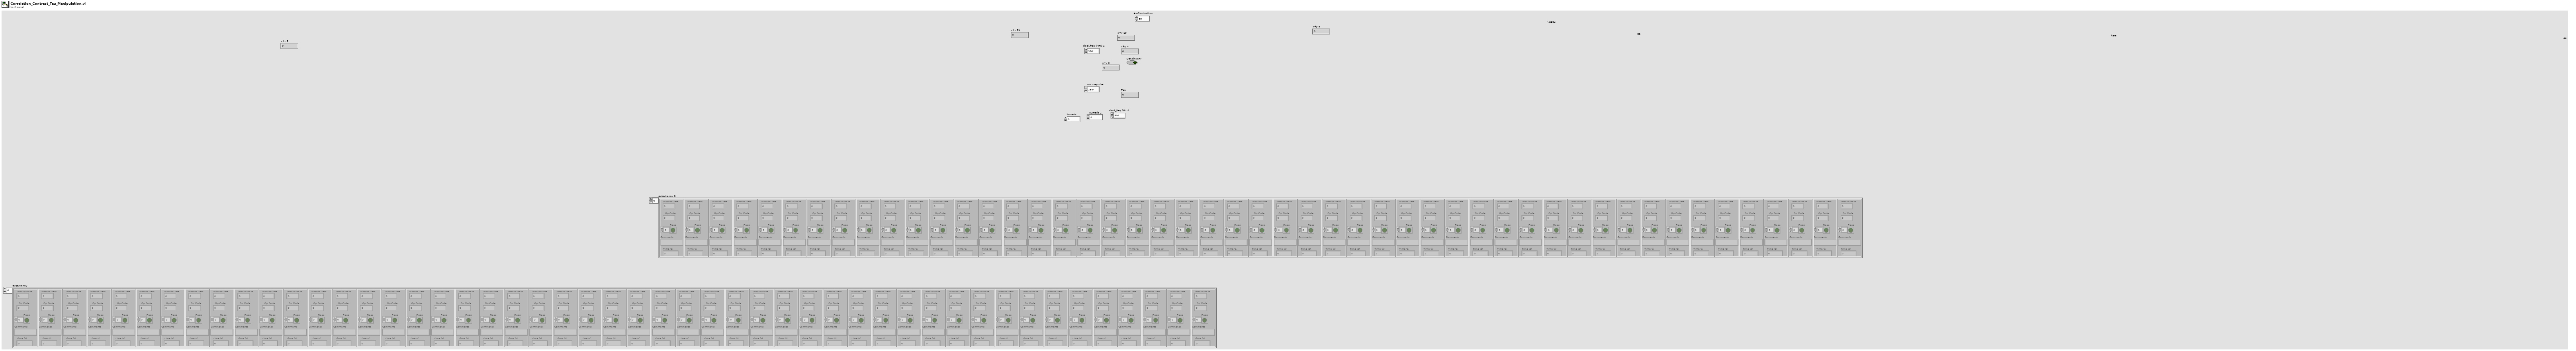
[diagram p1: front panel]
types:
  T1 = cluster{"Instruct Data":i32, "Op Code":i32, "Flags":bool[], "Comments":string, "Time (s)":dbl}[]
  T2 = typedef "DialogTypeEnum.ctl" = enum16{"no dialog", "OK message", "continue or stop message", "auto error handling dialog", "OK message + warnings", "continue/stop + warnings"}
  T3 = enum16{"Pulse Program", "Frequency Registers", "TX Phase Registers", "RX Phase Registers"}
  T4 = cluster{"Instruct Data":i32, "Op Code":i32, "Flags":bool[], "Comments":string, "Time (s)":dbl}
  T5 = cluster{"Instruct Data":i32, "Op Code":i32, "Flags":bool[], "Comments":string, dbl}
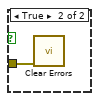
[diagram p3: hidden frame]
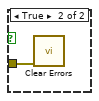
[diagram p4: hidden frame]
diagram:
  n1 = case shown="True" "Dont invert?" {
    tunnel: "Instructions" -> [w6 w109]
    tunnel: "# of Instructions" -> [w8 w108]
    tunnel: "# of Instructions" -> [w7 w107]
    tunnel: "MW Step Size" -> [w10 w106]
    tunnel: [w9 w105] -> w1
    frame False {
      n2 = flat-sequence {
        tunnel: w8 -> [w18]
        tunnel: [w13] -> _
        tunnel: w10 -> [w17]
        tunnel: [w14] -> w9
        tunnel: w7 -> [w13]
        tunnel: w6 -> [w12]
        frame #0 {
          # "DARk"
          # "tau"
          n3 = Wait (ms)(milliseconds to wait=u32 10) -> ()  [unwired: 1 out]
          n4 = property on="Instructions" class="Arr (strict)"(error in=errorcluster {"status"=FALSE, "code"=0, "source"=""} ("error in (no error)"), "Number of Columns"=w13) -> (error out=w59:errorcluster)  [unwired: 1 in, 1 out]
          n5 = global read "SpinCore_API_file_location.vi" "Path"() -> (w60:path)
          n6 = Reshape Array "Reshape Array"(w12, w18) -> (w65:T1)
          n7 = for {
            N: "Numeric 2" -> [_]
            tunnel: [w96] -> w61
            tunnel: [w95] -> w16 mode=indexing
            tunnel: w17 -> [w95]
            i -> [w97]
            n8 = Multiply(x=w95, y=w97) -> (x*y=w96:dbl)
          }
          n9 = Index Array "Index Array"(array=w65, index=22) -> (element=w64:T4)
          n10 = Unbundle By Name "Unbundle By Name"(w64) -> ("Instruct Data"=w70:i32, "Op Code"=w69:i32, "Flags"=w68:bool[], "Comments"=w67:string, "Time (s)"=w66:dbl)
          n11 = call "pb_init.vi"("error in (no error)"=w59, "path in"=w60) -> ("error out"=w58:errorcluster, "path out"=w57:path)  [unwired: 8 in]
          n12 = call "pb_core_clock.vi"("error in (no error)"=w58, "clock_freq (MHz)"="clock_freq (MHz) 2", "path in"=w57) -> ("error out"=w74:errorcluster, "path out"=w75:path)  [unwired: 7 in]
          n13 = Add(x=w66, y=w61) -> (x+y=w14:dbl)
          n14 = call "pb_start_programming.vi"("error in (no error)"=w74, "Device"=T3."Pulse Program", "path in"=w75) -> ("error out"=w81:errorcluster, "path out"=w85:path)  [unwired: 1 in, 6 out]
          n15 = Bundle("Instruct Data"=w70, "Op Code"=w69, "Flags"=w68, "Comments"=w67, w14) -> (w62:T5)  [unwired: 1 in]
          n16 = Replace Array Subset "Replace Array Subset"(array=w65, new element=w62, index=22) -> (w43:T1)
          n17 = for {
            N: "Numeric 2" -> [_]
            tunnel: [w93] -> w44
            tunnel: w16 -> [w92] mode=indexing
            i -> [w94]
            n18 = Multiply(x=w92, y=w94) -> (x*y=w93:dbl)
          }
          n19 = Index Array "Index Array"(array=w43, index=66) -> (element=w47:T4)
          n20 = Unbundle(w47) -> ("Instruct Data"=w53:i32, "Op Code"=w52:i32, "Flags"=w51:bool[], "Comments"=w50:string, "Time (s)"=w49:dbl)
          n21 = Add(x=w49, y=w44) -> (x+y=w48:dbl)
          "x+y 11" <- w48
          n22 = Bundle("Instruct Data"=w53, "Op Code"=w52, "Flags"=w51, "Comments"=w50, w48) -> (w45:T5)  [unwired: 1 in]
          n23 = Replace Array Subset "Replace Array Subset"(array=w43, new element=w45, index=66) -> (w31:T1)
          n24 = for {
            N: "Numeric 2" -> [_]
            tunnel: [w90] -> w32
            tunnel: w16 -> [w89] mode=indexing
            i -> [w91]
            n25 = Multiply(x=w89, y=w91) -> (x*y=w90:dbl)
          }
          n26 = Index Array "Index Array"(array=w31, index=46) -> (element=w35:T4)
          n27 = Unbundle(w35) -> ("Instruct Data"=w41:i32, "Op Code"=w40:i32, "Flags"=w39:bool[], "Comments"=w38:string, "Time (s)"=w37:dbl)
          n28 = for {
            N: "Numeric 2" -> [_]
            tunnel: [w87] -> w21
            tunnel: w16 -> [w86] mode=indexing
            i -> [w88]
            n29 = Multiply(x=w86, y=w88) -> (x*y=w87:dbl)
          }
          n30 = Subtract(x=w37, y=w32) -> (x-y=w36:dbl)
          "x+y 10" <- w36
          n31 = Bundle("Instruct Data"=w41, "Op Code"=w40, "Flags"=w39, "Comments"=w38, w36) -> (w33:T5)  [unwired: 1 in]
          n32 = Replace Array Subset "Replace Array Subset"(array=w31, new element=w33, index=46) -> (w20:T1)
          n33 = Index Array "Index Array"(array=w20, index=1) -> (element=w24:T4)
          n34 = Unbundle(w24) -> ("Instruct Data"=w30:i32, "Op Code"=w29:i32, "Flags"=w28:bool[], "Comments"=w27:string, "Time (s)"=w26:dbl)
          n35 = Subtract(x=w26, y=w21) -> (x-y=w25:dbl)
          "x+y 9" <- w25
          n36 = Bundle("Instruct Data"=w30, "Op Code"=w29, "Flags"=w28, "Comments"=w27, w25) -> (w22:T5)  [unwired: 1 in]
          n37 = Replace Array Subset "Replace Array Subset"(array=w20, new element=w22, index=1) -> (w11:T1)
          "output array 2" <- w11
          n38 = for {
            tunnel: w11 -> [w100] mode=indexing
            shift-right: [w102] -> w83
            shift-left: w85 -> [w103]
            shift-right: [w99] -> w80
            shift-left: w81 -> [w101]
            n39 = call "pb_inst_pbonly.vi"("error in (no error)"=w101, "PB Instruction"=w100, "path in"=w103) -> ("error out"=w99:errorcluster, "path out"=w102:path)  [unwired: 2 in, 5 out]
          }
          n40 = call "pb_stop_programming.vi"("error in (no error)"=w80, "path in"=w83) -> ("error out"=w79:errorcluster, "path out"=w84:path)  [unwired: 1 in, 7 out]
          n41 = call "pb_close.vi"("error in (no error)"=w79, "path in"=w84) -> ("error out"=w72:errorcluster)  [unwired: 9 out]
          n42 = call "General Error Handler MOD.vi"("type of dialog (OK msg:1)"=DialogTypeEnum."continue or stop message", "error in (no error)"=w72) -> ("STOP?"=w76:bool, "error out"=w77:errorcluster)  [unwired: 12 out]
          n43 = case shown="False" w76 {
            tunnel: w77 -> [_ w98]
            frame False {
            }
            frame True {
              n44 = call <vilib>:"Clear Errors.vi"("error in (no error)"=w98) -> ()  [unwired: 1 in, 6 out]
            }
          }
        }
        frame #1 {
          n45 = Wait (ms)(milliseconds to wait=u32 1) -> ()  [unwired: 1 out]
        }
      }
    }
    frame True {
      n46 = flat-sequence {
        tunnel: w109 -> [w117]
        tunnel: w108 -> [w116]
        tunnel: w107 -> [w115]
        tunnel: w106 -> [w114]
        tunnel: [w113] -> w105
        frame #0 {
          # "tau"
          n47 = Wait (ms)(milliseconds to wait=u32 10) -> ()  [unwired: 1 out]
          n48 = property on="Instructions" class="Arr (strict)"(error in=errorcluster {"status"=FALSE, "code"=0, "source"=""} ("error in (no error)"), "Number of Columns"=w115) -> (error out=w158:errorcluster)  [unwired: 1 in, 1 out]
          n49 = Reshape Array "Reshape Array"(w117, w116) -> (w164:T1)
          n50 = global read "SpinCore_API_file_location.vi" "Path"() -> (w159:path)
          n51 = for {
            N: "Numeric" -> [_]
            tunnel: [w195] -> w160
            tunnel: [w194] -> w112 mode=indexing
            tunnel: w114 -> [w194]
            i -> [w196]
            n52 = Multiply(x=w194, y=w196) -> (x*y=w195:dbl)
          }
          n53 = Index Array "Index Array"(array=w164, index=22) -> (element=w163:T4)
          n54 = Unbundle By Name "Unbundle By Name"(w163) -> ("Instruct Data"=w169:i32, "Op Code"=w168:i32, "Flags"=w167:bool[], "Comments"=w166:string, "Time (s)"=w165:dbl)
          n55 = call "pb_init.vi"("error in (no error)"=w158, "path in"=w159) -> ("error out"=w157:errorcluster, "path out"=w156:path)  [unwired: 8 in]
          n56 = call "pb_core_clock.vi"("error in (no error)"=w157, "clock_freq (MHz)"="clock_freq (MHz)", "path in"=w156) -> ("error out"=w173:errorcluster, "path out"=w174:path)  [unwired: 7 in]
          n57 = Add(x=w165, y=w160) -> (x+y=w113:dbl)
          n58 = call "pb_start_programming.vi"("error in (no error)"=w173, "Device"=T3."Pulse Program", "path in"=w174) -> ("error out"=w180:errorcluster, "path out"=w184:path)  [unwired: 1 in, 6 out]
          n59 = Bundle("Instruct Data"=w169, "Op Code"=w168, "Flags"=w167, "Comments"=w166, w113) -> (w161:T5)  [unwired: 1 in]
          n60 = Replace Array Subset "Replace Array Subset"(array=w164, new element=w161, index=22) -> (w142:T1)
          n61 = for {
            N: "Numeric" -> [_]
            tunnel: [w192] -> w143
            tunnel: w112 -> [w191] mode=indexing
            i -> [w193]
            n62 = Multiply(x=w191, y=w193) -> (x*y=w192:dbl)
          }
          n63 = Index Array "Index Array"(array=w142, index=66) -> (element=w146:T4)
          n64 = Unbundle By Name "Unbundle By Name"(w146) -> ("Instruct Data"=w152:i32, "Op Code"=w151:i32, "Flags"=w150:bool[], "Comments"=w149:string, "Time (s)"=w148:dbl)
          n65 = Add(x=w148, y=w143) -> (x+y=w147:dbl)
          "x+y 2" <- w147
          n66 = Bundle("Instruct Data"=w152, "Op Code"=w151, "Flags"=w150, "Comments"=w149, w147) -> (w144:T5)  [unwired: 1 in]
          n67 = Replace Array Subset "Replace Array Subset"(array=w142, new element=w144, index=66) -> (w130:T1)
          n68 = for {
            N: "Numeric" -> [_]
            tunnel: [w189] -> w131
            tunnel: w112 -> [w188] mode=indexing
            i -> [w190]
            n69 = Multiply(x=w188, y=w190) -> (x*y=w189:dbl)
          }
          n70 = Index Array "Index Array"(array=w130, index=66) -> (element=w134:T4)
          n71 = Unbundle By Name "Unbundle By Name"(w134) -> ("Instruct Data"=w140:i32, "Op Code"=w139:i32, "Flags"=w138:bool[], "Comments"=w137:string, "Time (s)"=w136:dbl)
          n72 = for {
            N: "Numeric" -> [_]
            tunnel: [w186] -> w120
            tunnel: w112 -> [w185] mode=indexing
            i -> [w187]
            n73 = Multiply(x=w185, y=w187) -> (x*y=w186:dbl)
          }
          n74 = Subtract(x=w136, y=w131) -> (x-y=w135:dbl)
          "x+y 3" <- w135
          n75 = Bundle("Instruct Data"=w140, "Op Code"=w139, "Flags"=w138, "Comments"=w137, w135) -> (w132:T5)  [unwired: 1 in]
          n76 = Replace Array Subset "Replace Array Subset"(array=w130, new element=w132, index=66) -> (w119:T1)
          n77 = Index Array "Index Array"(array=w119, index=1) -> (element=w123:T4)
          n78 = Unbundle By Name "Unbundle By Name"(w123) -> ("Instruct Data"=w129:i32, "Op Code"=w128:i32, "Flags"=w127:bool[], "Comments"=w126:string, "Time (s)"=w125:dbl)
          n79 = Subtract(x=w125, y=w120) -> (x-y=w124:dbl)
          "x+y 4" <- w124
          n80 = Bundle("Instruct Data"=w129, "Op Code"=w128, "Flags"=w127, "Comments"=w126, w124) -> (w121:T5)  [unwired: 1 in]
          n81 = Replace Array Subset "Replace Array Subset"(array=w119, new element=w121, index=1) -> (w110:T1)
          "output array" <- w110
          n82 = for {
            tunnel: w110 -> [w199] mode=indexing
            shift-right: [w201] -> w182
            shift-left: w184 -> [w202]
            shift-right: [w198] -> w179
            shift-left: w180 -> [w200]
            n83 = call "pb_inst_pbonly.vi"("error in (no error)"=w200, "PB Instruction"=w199, "path in"=w202) -> ("error out"=w198:errorcluster, "path out"=w201:path)  [unwired: 2 in, 5 out]
          }
          n84 = call "pb_stop_programming.vi"("error in (no error)"=w179, "path in"=w182) -> ("error out"=w178:errorcluster, "path out"=w183:path)  [unwired: 1 in, 7 out]
          n85 = call "pb_close.vi"("error in (no error)"=w178, "path in"=w183) -> ("error out"=w171:errorcluster)  [unwired: 9 out]
          n86 = call "General Error Handler MOD.vi"("type of dialog (OK msg:1)"=DialogTypeEnum."continue or stop message", "error in (no error)"=w171) -> ("STOP?"=w175:bool, "error out"=w176:errorcluster)  [unwired: 12 out]
          n87 = case shown="False" w175 {
            tunnel: w176 -> [_ w197]
            frame False {
            }
            frame True {
              n88 = call <vilib>:"Clear Errors.vi"("error in (no error)"=w197) -> ()  [unwired: 1 in, 6 out]
            }
          }
        }
        frame #1 {
          n89 = Wait (ms)(milliseconds to wait=u32 1) -> ()  [unwired: 1 out]
        }
      }
    }
  }
  "Tau" <- w1
